vi "DSS-Tests-golden_compare.vi"(8 "abs tol":dbl, 9 "rel tol":dbl=1e-12, 10 "golden":dbl[](array[numeric]), 11 "actual":dbl[](array[numeric])) -> (1 "max rel diff":dbl, 2 "message":string, 3 "pass":bool)   [LabVIEW 2020, in "DSS-Tests.lvlib"]
doc: "Compares an actual 1D DBL array with a golden one (sizes, then each element through DSS-Tests-golden_elements) and reports pass with a message naming the sizes, the failing count, the first failing index with both values and the max relative difference."
uses:
  DSS-Tests.lvlib
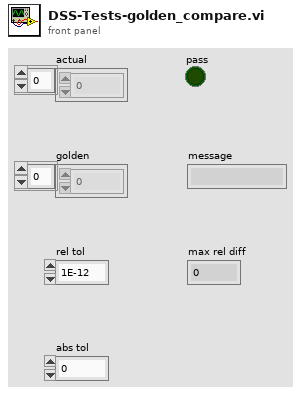
[diagram p1: front panel]
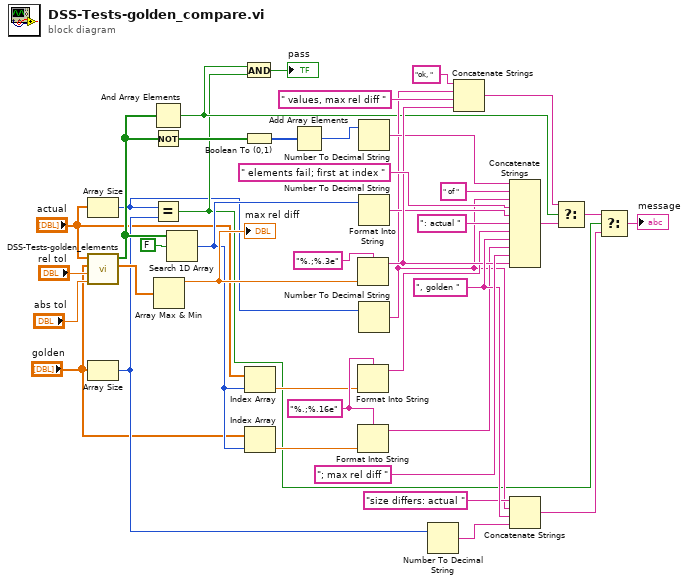
[diagram p0: block diagram]
diagram:
  w30 = ", golden " ("t golden")
  w20 = "%.;%.16e" ("value format")
  n1 = Array Size(array="actual") -> (size(s)=w5:i32)
  n2 = call "DSS-Tests-golden_elements.vi"("abs tol"="abs tol", "rel tol"="rel tol", "golden"="golden", "actual"="actual") -> ("rel diff"=w9:dbl[], "element ok"=w8:bool[])  [unwired: 6 in]
  n3 = Array Size(array="golden") -> (size(s)=w6:i32)
  n4 = And Array Elements(Boolean array=w8) -> (logical AND=w10:bool)
  n5 = Not(x=w8) -> (.not. x?=w12:bool[])
  n6 = Equal?(x=w5, y=w6) -> (x = y?=w7:bool)
  n7 = Array Max & Min(array=w9) -> (max value=w19:dbl)  [unwired: 3 out]
  "max rel diff" <- w19
  n8 = Search 1D Array(1D array=w8, element=FALSE ("false")) -> (index of element=w16:i32)  [unwired: 1 in]
  n9 = And(x=w10, y=w7) -> (x .and. y?=→"pass":bool)
  n10 = Boolean To (0,1)(Boolean=w12) -> (0, 1=w13:i16[])
  n11 = Index Array(array="actual", index=w16) -> (element=w17:dbl)
  n12 = Index Array(array="golden", index=w16) -> (element=w18:dbl)
  n13 = Add Array Elements(numeric array=w13) -> (sum=w14:i16)
  n14 = Format Into String(format string="%.;%.3e" ("rel format"), w19) -> (resulting string=w28:string)  [unwired: 2 in, 1 out]
  n15 = Format Into String(format string=w20, w17) -> (resulting string=w26:string)  [unwired: 2 in, 1 out]
  n16 = Format Into String(format string=w20, w18) -> (resulting string=w27:string)  [unwired: 2 in, 1 out]
  n17 = Number To Decimal String(number=w14) -> (decimal integer string=w24:string)  [unwired: 1 in]
  n18 = Number To Decimal String(number=w16) -> (decimal integer string=w25:string)  [unwired: 1 in]
  n19 = Number To Decimal String(number=w5) -> (decimal integer string=w22:string)  [unwired: 1 in]
  n20 = Number To Decimal String(number=w6) -> (decimal integer string=w23:string)  [unwired: 1 in]
  n21 = Concatenate Strings("ok, " ("t ok"), w22, " values, max rel diff " ("t values"), w28) -> (w39:string)
  n22 = Concatenate Strings(w24, " of " ("t of"), w22, " elements fail; first at index " ("t fail"), w25, ": actual " ("t actual"), w26, w30, w27, "; max rel diff " ("t maxrel"), w28) -> (w38:string)
  n23 = Concatenate Strings("size differs: actual " ("t size"), w22, w30, w23) -> (w37:string)
  n24 = Select(t=w39, s=w10, f=w38) -> (s? t:f=w40:string)
  n25 = Select(t=w40, s=w7, f=w37) -> (s? t:f=→"message":string)
